vi "Create GUI Element.vi"(8 "error in (no error)":errorcluster, 10 "Highlight":bool, 11 "Schedule Cell in":refnum<class "Schedule Cell.lvclass">) -> (0 "error out":errorcluster, 2 "RUN properties":T1={"Background Color"=16777226, "Number of cycles"=1, "Single RUN"={"Script Name"="", "Parameters"=[], "FPGA Name"=""}, "Quality check"=FALSE, "Cell Type"=""} {"Number of cycles" min=1}, 3 "Schedule Cell out":refnum<class "Schedule Cell.lvclass">)   [LabVIEW 2020, in "Run Utilities.lvlib" / "Schedule Cell.lvclass"]
doc: "Create a GUI object with information about the Schedule Cell"
uses:
  Schedule Cell.lvclass
  Cell - GUI.ctl
  Run Instance/Run Instance - GUI.ctl
  Run Instance/Run Instance.lvclass
  Schedule Cell.lvclass/Schedule Cell.ctl
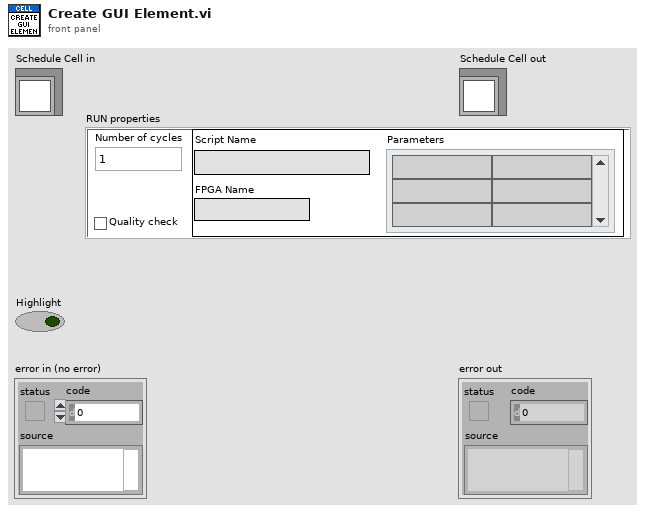
[diagram p1: front panel]
types:
  T1 = typedef "Run Utilities.lvlib/Schedule Cell.lvclass/Cell - GUI.ctl" = cluster{"Background Color":u32, "Number of cycles":u32, "Single RUN":T2, "Quality check":bool, "Cell Type":string}
  T2 = typedef "Run Utilities.lvlib/Run Instance.lvclass/Run Instance - GUI.ctl" = cluster{"Script Name":string, "Parameters":string[][], "FPGA Name":string}
  T3 = cluster{"Name":string, "Comparison":string, "Value":string}[]
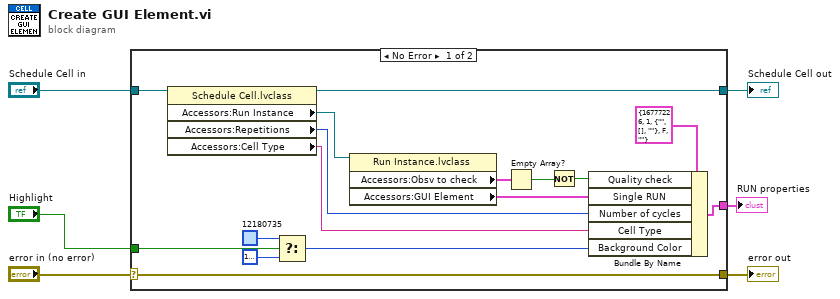
[diagram p0: block diagram]
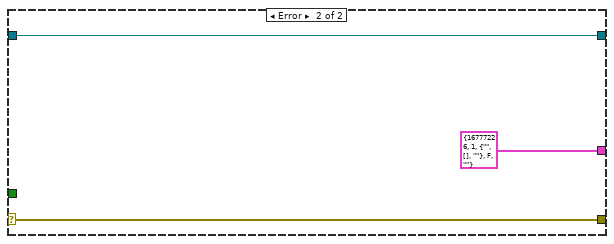
[diagram p2: hidden frame]
diagram:
  n1 = case shown="No Error" "error in (no error)" {
    selector: "error in (no error)" -> [w22 w25]
    tunnel: [w22 w25] -> w5
    tunnel: [w14 w24] -> w3
    tunnel: "Schedule Cell in" -> [w15 w24]
    tunnel: [w20 T1 {"Background Color"=16777226, "Number of cycles"=1, "Single RUN"={"Script Name"="", "Parameters"=[], "FPGA Name"=""}, "Quality check"=FALSE, "Cell Type"=""} ("RUN properties")] -> w2
    tunnel: "Highlight" -> [w7 _]
    frame No Error {
      n2 = property class="Schedule Cell.lvclass"(reference=w15) -> (reference out=w14:refnum<class "Schedule Cell.lvclass">, "Accessors:Run Instance"=w13:refnum<class "Run Instance.lvclass">, "Accessors:Repetitions"=w12:u32, "Accessors:Cell Type"=w11:string)  [unwired: 1 in, 1 out]
      n3 = Select(t=u32 12180735 ("Bcg Color"), s=w7, f=u32 16777226 ("Background Color")) -> (s? t:f=w8:u32)
      n4 = property class="Run Instance.lvclass"(reference=w13) -> ("Accessors:Obsv to check"=w19:T3, "Accessors:GUI Element"=w18:T2)  [unwired: 1 in, 2 out]
      n5 = Empty Array?(array=w19) -> (empty?=w17:bool)
      n6 = Not(x=w17) -> (.not. x?=w16:bool)
      n7 = Bundle By Name(cluster=T1 {"Background Color"=16777226, "Number of cycles"=1, "Single RUN"={"Script Name"="", "Parameters"=[], "FPGA Name"=""}, "Quality check"=FALSE, "Cell Type"=""} ("RUN properties"), "Quality check"=w16, "Single RUN"=w18, "Number of cycles"=w12, "Cell Type"=w11, "Background Color"=w8) -> (w20:T1)
    }
    frame Error {
    }
  }
  "error out" <- w5
  "Schedule Cell out" <- w3
  "RUN properties" <- w2
